vi "Close MeasurementLink Session.vi"(8 "error in":errorcluster, 9 "initialize and close session behavior":T1, 10 "session in":variant, 11 "session factory in":refnum<class "Session Factory.lvclass">) -> (0 "error out":errorcluster)   [LabVIEW 2021, in "Session Management niDAQmx.lvlib" / "Session Factory.lvclass"]
doc: "Closes the local session. If the session represents a remote session, <b>initialize and close session behavior</b> determines whether closing the local session closes the server session or detaches from the server session."
uses:
  Session Factory.lvclass
  <vilib>/Plug-In SDKs/Sessions/Instrument/ISession Factory/Initialize and Close Session Behavior.ctl
  Session Factory.lvclass/Session Factory.ctl
  NI DAQmx Client/RPC Messages/nidaqmx_grpc_ClearTaskRequest.ctl
  NI DAQmx Client/RPC Messages/nidevice_grpc_Session.ctl
  NI DAQmx Client/RPC Messages/nidevice_grpc_Session_session/nidevice_grpc_Session_session.lvclass
  NI DAQmx Client/NI_DAQmx_client.lvlib
  <vilib>/Plug-In SDKs/Sessions/Instrument/ISession Factory/ISession Factory.lvclass
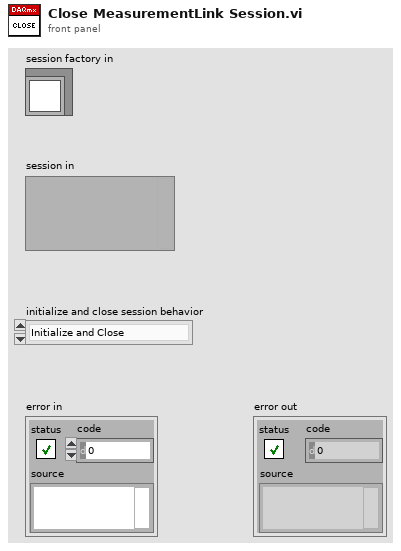
[diagram p1: front panel]
types:
  T1 = typedef "NI Session Management Instrument.lvlib/ISession Factory.lvclass/Initialize and Close Session Behavior.ctl" = enum16{"Initialize and Close", "Attach and Detach", "Initialize and Detach", "Attach and Close"}
  T2 = typedef "grpc-lvsupport-release.lvlib/grpcId.ctl" = u64
  T3 = typedef "NI_DAQmx_client.lvlib/nidaqmx_grpc_ClearTaskRequest.ctl" = cluster{"task":T4}
  T4 = typedef "NI_DAQmx_client.lvlib/nidevice_grpc_Session.ctl" = cluster{"nidevice_grpc_Session_session":refnum<class "nidevice_grpc_Session_session.lvclass">}
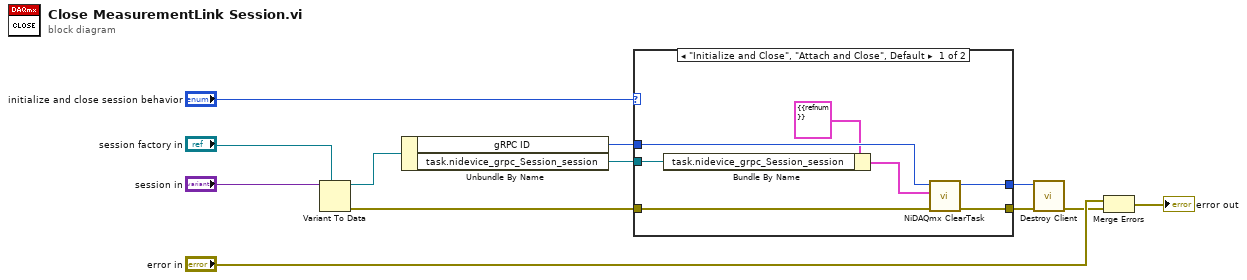
[diagram p0: block diagram]
diagram:
  n1 = Variant To Data(type="session factory in", Variant="session in") -> (data=w4:refnum<class "Session Factory.lvclass">, error out=w5:errorcluster)  [unwired: 1 in]
  n2 = Unbundle By Name(w4) -> ("gRPC ID"=w9:T2, "task.nidevice_grpc_Session_session"=w8:refnum<class "nidevice_grpc_Session_session.lvclass">)
  n3 = case shown="\"Initialize and Close\", \"Attach and Close\", Default" "initialize and close session behavior" {
    tunnel: w5 -> [w19 w20]
    tunnel: [w18 w20] -> w6
    tunnel: w9 -> [w17 w21]
    tunnel: w8 -> [w15 _]
    tunnel: [w13 w21] -> w7
    frame "Initialize and Close", "Attach and Close", Default {
      n4 = Bundle By Name(cluster=T3 {"task"={"nidevice_grpc_Session_session"=refnum}} ("Request Data"), "task.nidevice_grpc_Session_session"=w15) -> (w14:T3)
      n5 = call "NiDAQmx ClearTask.vi"("error in"=w19, "Request Data"=w14, "gRPC ID"=w17) -> ("error out"=w18:errorcluster, "gRPC ID out"=w13:T2)  [unwired: 6 in, 1 out]
    }
    frame "Attach and Detach", "Initialize and Detach" {
    }
  }
  n6 = call "Destroy Client.vi"("error in"=w6, "gRPC ID"=w7) -> ("error out"=w2:errorcluster)  [unwired: 9 in]
  n7 = Merge Errors("error in", w2) -> (→"error out":errorcluster)
